vi "View Waveform.vi"() -> ()   [LabVIEW 2012]
panel:
  out "Array Zize":i32
  out "File Path":path
  out "Waveform Graph":waveform(dbl)(graph)
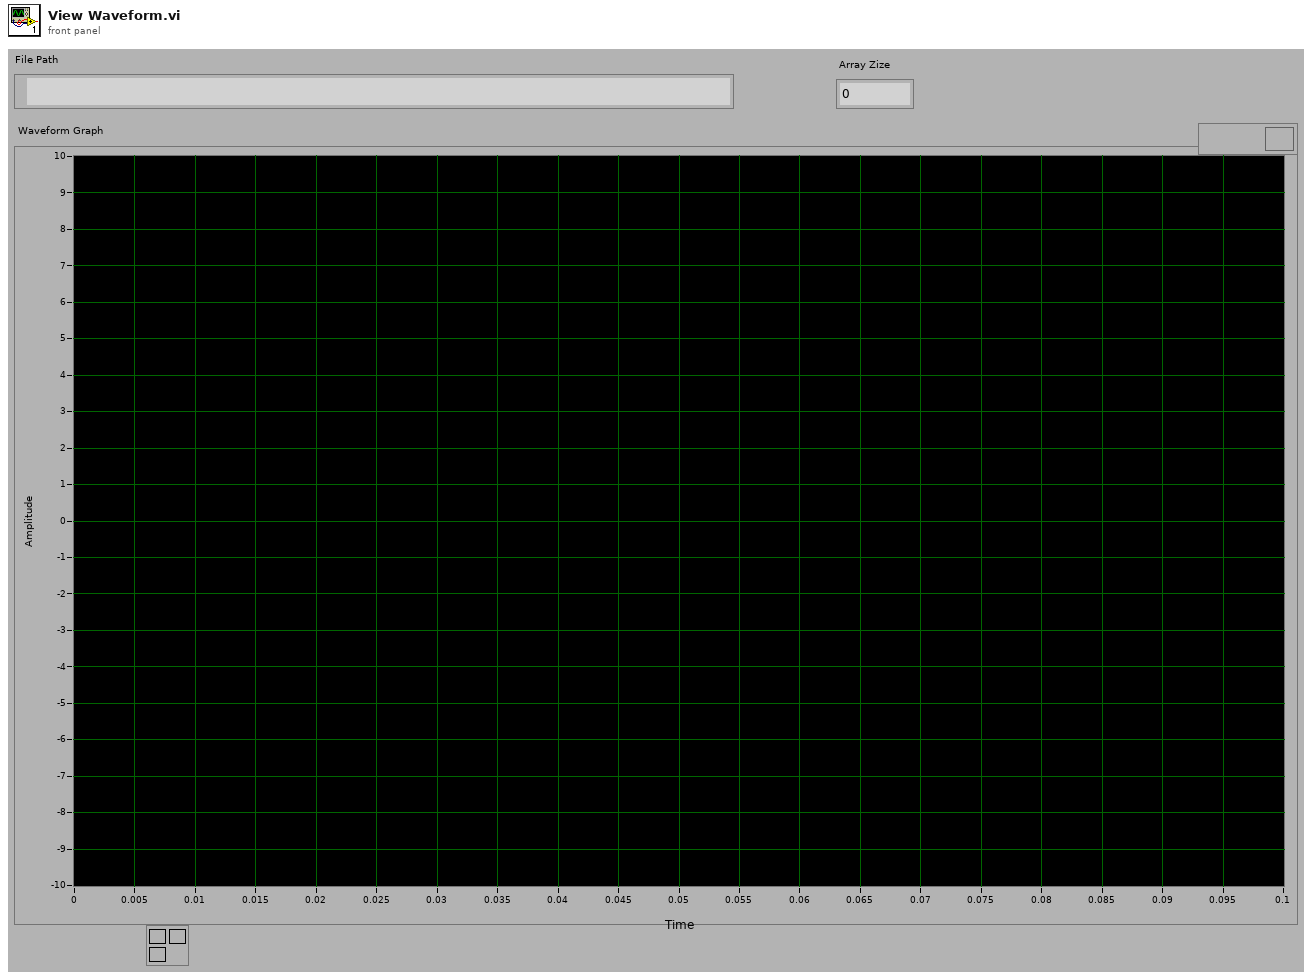
[diagram p1: front panel]
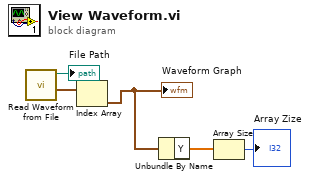
[diagram p0: block diagram]
diagram:
  n1 = call <vilib>:"Read Waveform from File.vi"() -> ("all waveforms in record"=w5:waveform(dbl)[], "new file path (Not A Path if cancelled)"=→"File Path":path)  [unwired: 6 in, 2 out]
  n2 = Index Array(array=w5) -> (element=w1:waveform(dbl))  [unwired: 1 in]
  "Waveform Graph" <- w1
  n3 = Unbundle By Name(w1) -> ("Y"=w3:dbl[])
  n4 = Array Size(array=w3) -> (size(s)=→"Array Zize":i32)
